vi "resources templates list.vi"(8 "error in":errorcluster, 11 "message json":string) -> (0 "error out":errorcluster, 3 "response":string)   [LabVIEW 2020, in "MCP Server.lvlib"]
doc: "Handles the JSON-RPC method resources/templates/list. This server has no resource templates, so the answer is an empty resourceTemplates array."
uses:
  MCP Server.lvlib
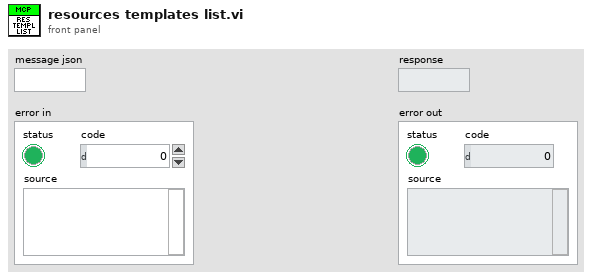
[diagram p1: front panel]
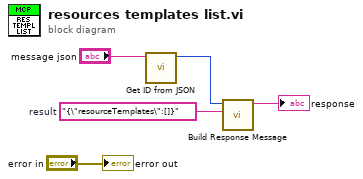
[diagram p0: block diagram]
diagram:
  w3 = "{\"resourceTemplates\":[]}"  # result
  n1 = call "Get ID from JSON.vi"("message json"="message json") -> ("Data out"=w4:i32)  [unwired: 10 in]
  n2 = call "Build Response Message.vi"("Result content"=w3, "message id in"=w4) -> ("MCP message out"=→"response":string)  [unwired: 8 in, 1 out]
  "error out" <- "error in"
